vi "Debug Interface.vi"() -> ()   [LabVIEW 2013]
panel:
  in  "stop":bool
  # "This VI does nothing except provide an accessible VI\nin the 'MxLVProvider\" application instance.  By\ndoing \"File >> New\" from this VI's window, you can\ncreate a blank VI in the provider application instance.\n\nYou can then put other provider subVIs on the block diagram\nof the new VI, and when you open them you'll be interacting\nwith the subVI instance _inside_ the provider app instance.\n\nThis allows you to probe/trace live provider VIs, which you\notherwise can't get to."
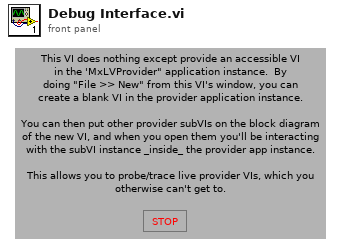
[diagram p1: front panel]
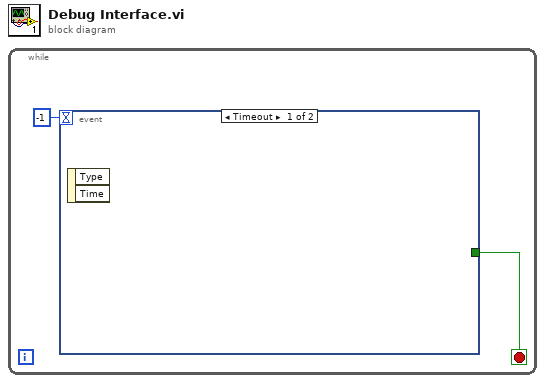
[diagram p0: block diagram]
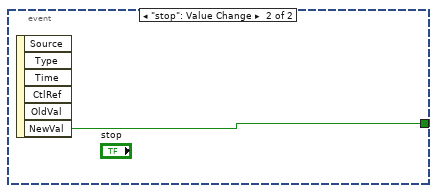
[diagram p2: hidden frame]
diagram:
  n1 = while {
    stop <- w2 stop-if-true
    n2 = event shown="[0] Timeout" {
      selector: _ -> [_ _]
      dyn-events: _ -> [_ _]
      timeout: -1 -> [_ _]
      tunnel: [_ w3] -> w2
      event Timeout {
        n3 = event-data() -> ()  [unwired: 1 in, 2 out]
      }
      event "stop": Value Change {
        n4 = event-data() -> ("NewVal"=w3:bool)  [unwired: 1 in, 5 out]
      }
    }
  }
